vi "detect controller.vi"(6 "Network Adapters":bool caption="network adapters (F)", 8 "error in":errorcluster, 11 "controller in":refnum<class "Controller.lvclass">) -> (0 "error out":errorcluster, 3 "controller out":refnum<class "Controller.lvclass">)   [LabVIEW 2014, in "SMI.lvlib" / "Controller.lvclass"]
uses:
  Controller.lvclass
  write secondary network adapters.vi
  write primary network adapter.vi
  write device information.vi
  write system hardware ref.vi
  Device/write device class.vi
  Device/write serial number.vi
  Device/write product ID.vi
  Device/write product name.vi
  Device/write vendor name.vi
  SysCfg Device/write system session.vi
  SysCfg Device/read system session.vi
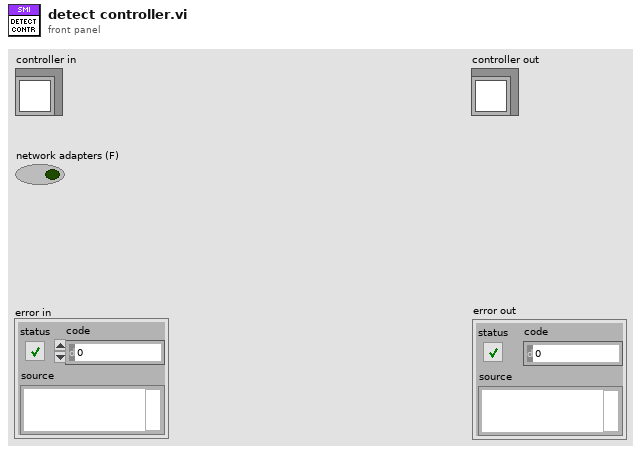
[diagram p1: front panel]
types:
  T1 = typedef "SMI.lvlib/Controller.lvclass/controller information.ctl" = cluster{"system session":refnum<data-value>, "system hardware ref":refnum<data-value>, "vendor name":string, "product name":string, "product ID":u16, "serial number":string, "device information":T2, "primary network adapter":T3, "secondary network adapters":T3[]}
  T2 = typedef "SMI.lvlib/Controller.lvclass/device information.ctl" = cluster{"resource":string, "device class":string, "system start time":timestamp, "current time":timestamp, "time zone":string, "firmware revision":string, "image title":string, "image version":string, "system status":string}
  T3 = typedef "SMI.lvlib/Controller.lvclass/network adapter settings.ctl" = cluster{"IP address":string, "MAC address":string, "IP address request mode":u32, "subnet mask":string, "gateway":string, "DNS server":string, "adapter mode":u32, "adapter type":u32}
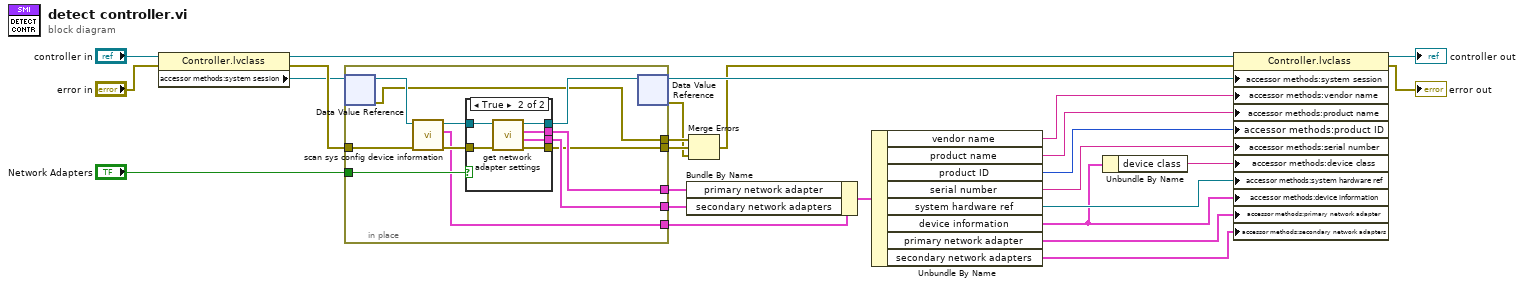
[diagram p0: block diagram]
diagram:
  n1 = property class="Controller.lvclass"(reference="controller in", error in="error in") -> (reference out=w15:refnum<class "Controller.lvclass">, error out=w20:errorcluster, "accessor methods:system session"=w14:refnum<data-value>)
  n2 = in-place {
    in-place-border: "Network Adapters" -> [w37]
    in-place-border: [w34] -> w25
    in-place-border: [w33] -> w24
    in-place-border: [w32] -> w23
    in-place-border: w20 -> [w28]
    in-place-border: [w29] -> w8
    in-place-border: [w27] -> w9
    n3 = in-place-dvr #1(w14) -> (w31:refnum<k21>, w27:errorcluster)
    n4 = call "scan sys config device information.vi"("error in"=w28, "system session in"=w31) -> ("error out"=w35:errorcluster, "controller information"=w33:T1, "system session out"=w36:refnum<k21>)  [unwired: 7 in]
    n5 = case shown="True" w37 {
      tunnel: w36 -> [w39 w45]
      tunnel: w35 -> [w38 w44]
      tunnel: [_ w43] -> w34
      tunnel: [w39 w42] -> w30
      tunnel: [w38 w41] -> w29
      tunnel: [_ w40] -> w32
      frame False {
      }
      frame True {
        n6 = call "get network adapter settings.vi"("error in"=w44, "system session in"=w45) -> ("error out"=w41:errorcluster, "secondary network adapters"=w40:T3[], "primary network adapter"=w43:T3, "system session out"=w42:refnum<k21>)  [unwired: 6 in]
      }
    }
    n7 = in-place-dvr #1(w30) -> (w12:refnum<data-value>, w7:errorcluster)
  }
  n8 = Bundle By Name(cluster=w24, "primary network adapter"=w25, "secondary network adapters"=w23) -> (w19:T1)
  n9 = Merge Errors(w9, w8, w7) -> (w10:errorcluster)
  n10 = Unbundle By Name(w19) -> ("vendor name"=w13:string, "product name"=w18:string, "product ID"=w17:u16, "serial number"=w16:string, "system hardware ref"=w6:refnum<data-value>, "device information"=w5:T2, "primary network adapter"=w4:T3, "secondary network adapters"=w3:T3[])
  n11 = Unbundle By Name(w5) -> ("device class"=w11:string)
  n12 = property class="Controller.lvclass"(reference=w15, error in=w10, "accessor methods:system session"=w12, "accessor methods:vendor name"=w13, "accessor methods:product name"=w18, "accessor methods:product ID"=w17, "accessor methods:serial number"=w16, "accessor methods:device class"=w11, "accessor methods:system hardware ref"=w6, "accessor methods:device information"=w5, "accessor methods:primary network adapter"=w4, "accessor methods:secondary network adapters"=w3) -> (reference out=→"controller out":refnum<class "Controller.lvclass">, error out=→"error out":errorcluster)
